vi "Init.vi"(8 "error in (no error)":errorcluster, 11 "bt_System in":refnum<class "bt_System.lvclass">) -> (0 "error out":errorcluster, 3 "bt_System out":refnum<class "bt_System.lvclass">)   [LabVIEW 2021, in "BT.lvlib" / "bt_System.lvclass"]
uses:
  bt_System.lvclass
  bt_System.lvclass/bt_System.ctl
  Support/Nodes/abs_Node/Status.ctl
  Support/Execution Engine.vi
  Support/Nodes/abs_Node/bt_Node.lvclass
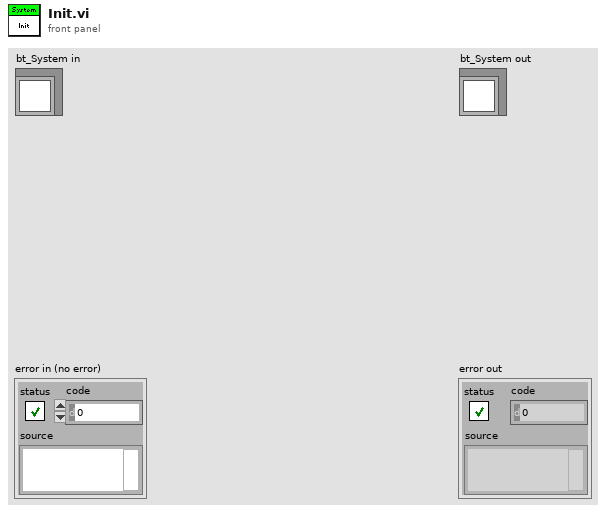
[diagram p1: front panel]
types:
  T1 = typedef "BT.lvlib/bt_Node.lvclass/Status.ctl" = enum16{"Success", "Failure", "Running"}
  T2 = typedef "Rendezvous RefNum" = refnum<k1>
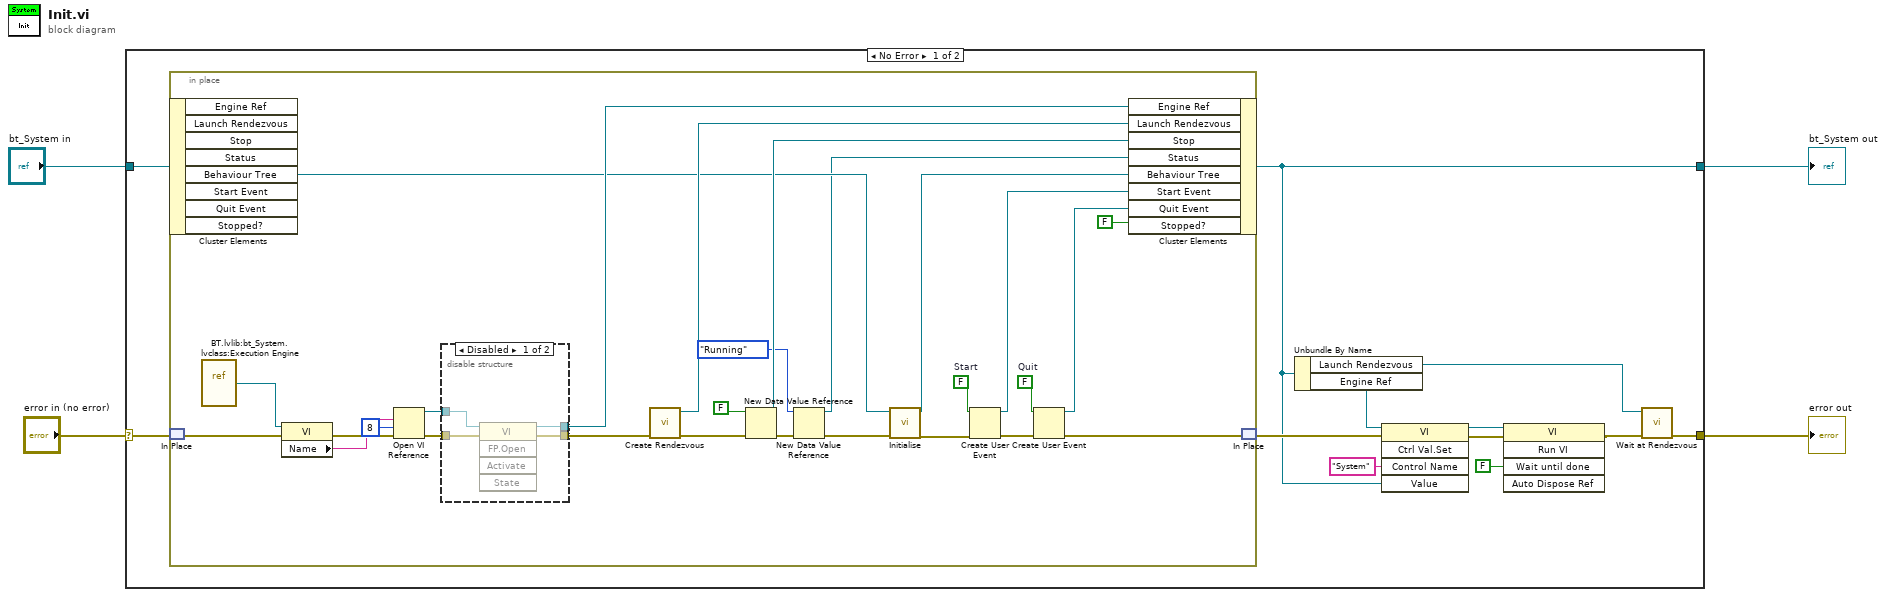
[diagram p0: block diagram]
diagram:
  n1 = case shown="No Error" "error in (no error)" {
    selector: "error in (no error)" -> [w16 w51]
    tunnel: [w6 w51] -> w3
    tunnel: [w12 w50] -> w1
    tunnel: "bt_System in" -> [w15 w50]
    frame No Error {
      n2 = in-place {
        w23 = FALSE  # Quit
        w24 = FALSE  # Start
        n3 = in-place-cluster #1(w15) -> ("Behaviour Tree"=w29:refnum<class "bt_Node.lvclass">)  [unwired: 7 out]
        n4 = in-place-match #2(w16) -> (w35:errorcluster)
        n5 = vi-ref "BT.lvlib:bt_System.lvclass:Execution Engine.vi"() -> (w42:refnum<vi>)
        n6 = property class="VI"(reference=w42, error in=w35) -> (error out=w43:errorcluster, "Name"=w41:string)  [unwired: 1 out]
        n7 = Open VI Reference(vi path=w41, options=8, error in (no error)=w43) -> (vi reference=w39:refnum<vi>, error out=w38:errorcluster)  [unwired: 3 in]
        n8 = disable-structure shown="Disabled" {
          disable-tunnel: w39 -> [w47 w49]
          disable-tunnel: w38 -> [w46 w48]
          disable-tunnel: [w45 w49] -> w30
          disable-tunnel: [w44 w48] -> w31
          frame Disabled {
            n9 = invoke class="VI" method="FP.Open"(reference=w47, error in=w46) -> (reference out=w45:refnum<vi>, error out=w44:errorcluster)  [unwired: 3 in, 3 out]
          }
          frame Enabled {
          }
        }
        n10 = call <vilib>:"Create Rendezvous.vi"("error in (no error)"=w31) -> ("error out"=w34:errorcluster, "rendezvous"=w37:T2)  [unwired: 4 in, 1 out]
        n11 = New Data Value Reference(data value=FALSE, error in=w34) -> (data value reference=w33:refnum<data-value>, error out=w28:errorcluster)
        n12 = New Data Value Reference(data value=Status."Running" ("y"), error in=w28) -> (data value reference=w26:refnum<data-value>, error out=w27:errorcluster)
        n13 = call-dynamic "Initialise.vi"("error in (no error)"=w27, "Node in"=w29) -> ("error out"=w22:errorcluster, "Node out"=w36:refnum<class "bt_Node.lvclass">)  [unwired: 8 in]
        n14 = Create User Event(user event datatype=w24, error in=w22) -> (user event=w21:refnum<user-event>, error out=w19:errorcluster)
        n15 = Create User Event(user event datatype=w23, error in=w19) -> (user event=w20:refnum<user-event>, error out=w17:errorcluster)
        n16 = in-place-cluster #1("Engine Ref"=w30, "Launch Rendezvous"=w37, "Stop"=w33, "Status"=w26, "Behaviour Tree"=w36, "Start Event"=w21, "Quit Event"=w20, "Stopped?"=FALSE) -> (w12:refnum<class "bt_System.lvclass">)
        n17 = in-place-match #2(w17) -> (w13:errorcluster)
      }
      n18 = Unbundle By Name(w12) -> ("Launch Rendezvous"=w5:T2, "Engine Ref"=w11:refnum<vi>)
      n19 = invoke class="VI" method="Ctrl Val.Set"(reference=w11, error in=w13, "Control Name"="System", "Value"=w12) -> (reference out=w8:refnum<vi>, error out=w9:errorcluster)  [unwired: 1 in, 3 out]
      n20 = invoke class="VI" method="Run VI"(reference=w8, error in=w9, "Wait until done"=FALSE ("Wait Until Done")) -> (error out=w7:errorcluster)  [unwired: 2 in, 4 out]
      n21 = call <vilib>:"Wait at Rendezvous.vi"("error in (no error)"=w7, "rendezvous"=w5) -> ("error out"=w6:errorcluster)  [unwired: 3 in, 2 out]
    }
    frame Error {
    }
  }
  "error out" <- w3
  "bt_System out" <- w1
